vi "Unflatten pcap CAN to XNET CAN.vi"(6 "Offset in":i32, 8 "error in (no error)":errorcluster, 10 "pcap CAN DATA in":u8[](array[numeric]), 11 "XNET_CAN_RW in":refnum<class "XNET CAN RW.lvclass">) -> (0 "error out":errorcluster, 1 "XNET CAN Data":T1[](array[typedef]) {"payload" format="%x"; "timestamp" format="%<%.7X\n%x>T"; "type" items=["CAN Data"=0, "CAN Remote"=1, "CAN Bus Error"=2, "CAN 2.0 Data"=8, "CAN FD Data"=16, "CAN FD+BRS Data"=24, "J1939 Data"=192, "Delay"=224, "Log Trigger"=225, "Start Trigger"=226]; "identifier" format="%x"}, 2 "pcap CAN DATA out":u8[](array[numeric]), 3 "XNET_CAN_RW out":refnum<class "XNET CAN RW.lvclass">, 4 "Offset out":i32, 5 "Number Filtered":u32)   [LabVIEW 2021, in "XNET CAN RW.lvclass"]
uses:
  XNET CAN RW.lvclass
  <vilib>/xnet/xnet.llb/XNET Frame CAN.ctl
  <vilib>/xnet/xnet.llb/XNET Frame Type CAN.ctl
  C:/Program Files/National Instruments/LabVIEW 2021/vi.lib/CIF Foundation/CIF CAN RW Core/CAN_RW_CORE.lvclass
  <vilib>/CIF Foundation/CIF CAN RW Core/CAN_RW_CORE.lvclass/CAN_RW_CORE.ctl
  <vilib>/CIF Foundation/CIF PCAP Parse and Build/pcap_Parse_Build_CIF.lvclass/pcap_Parse_Build_CIF.ctl
  <vilib>/CIF Foundation/CIF CAN RW Core/Accessors/Read pcap class.vi
  <vilib>/CIF Foundation/CIF CAN RW Core/Accessors/Write pcap class.vi
  <vilib>/CIF Foundation/CIF PCAP Parse and Build/Data Accessors/Write Offset.vi
  <vilib>/CIF Foundation/CIF Utilities/Time/System Time/TAI Time to LabVIEW Time.vi
  <vilib>/CIF Foundation/CIF PCAP Parse and Build/Parse/Unflatten Packet Header.vi
  <vilib>/CIF Foundation/CIF Utilities/DataTypes/Flatten Unflatten/Unflatten U32.vi
  <vilib>/CIF Foundation/CIF PCAP Parse and Build/Utilities/Add Error.vi
  <vilib>/CIF Foundation/CIF PCAP Parse and Build/Utilities/Add Error Core.vi
  <vilib>/CIF Foundation/CIF PCAP Parse and Build/pcap_Parse_Build_CIF.lvclass
  <vilib>/CIF Foundation/CIF CAN RW Core/CAN_RW_CORE.lvclass
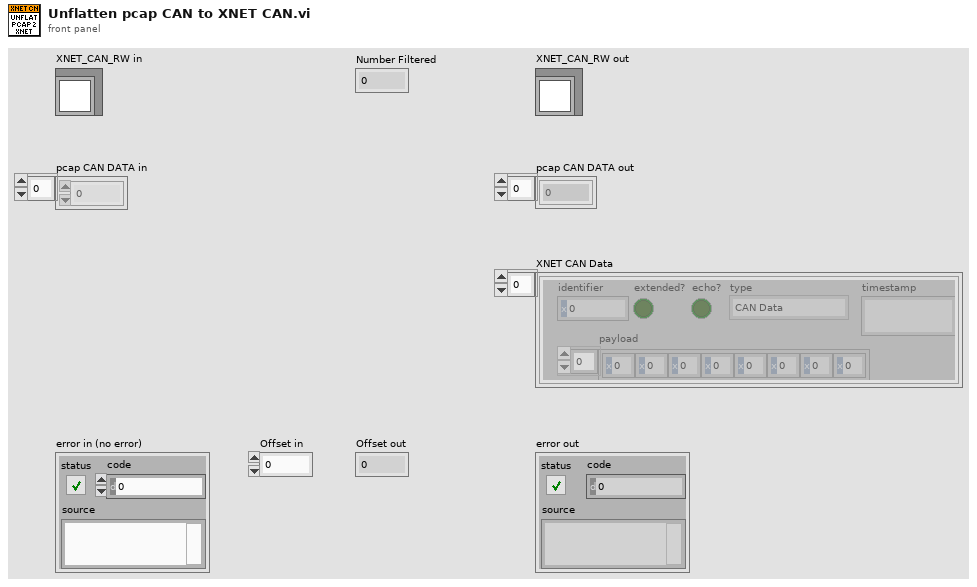
[diagram p1: front panel]
types:
  T1 = typedef "XNET Frame CAN.ctl" = cluster{"timestamp":timestamp, "payload":u8[], "identifier":u32, "type":T2, "extended?":bool, "echo?":bool}
  T2 = typedef "XNET Frame Type CAN.ctl" = u8
  T3 = typedef "pcap_Parse_Build_CIF.lvclass/Socket CAN Header.ctl" = cluster{"CANID and Flags":u32, "Payload Length":u8, "FD Flags":u8, "RSVD":u8, "Len8 DLC":u8}
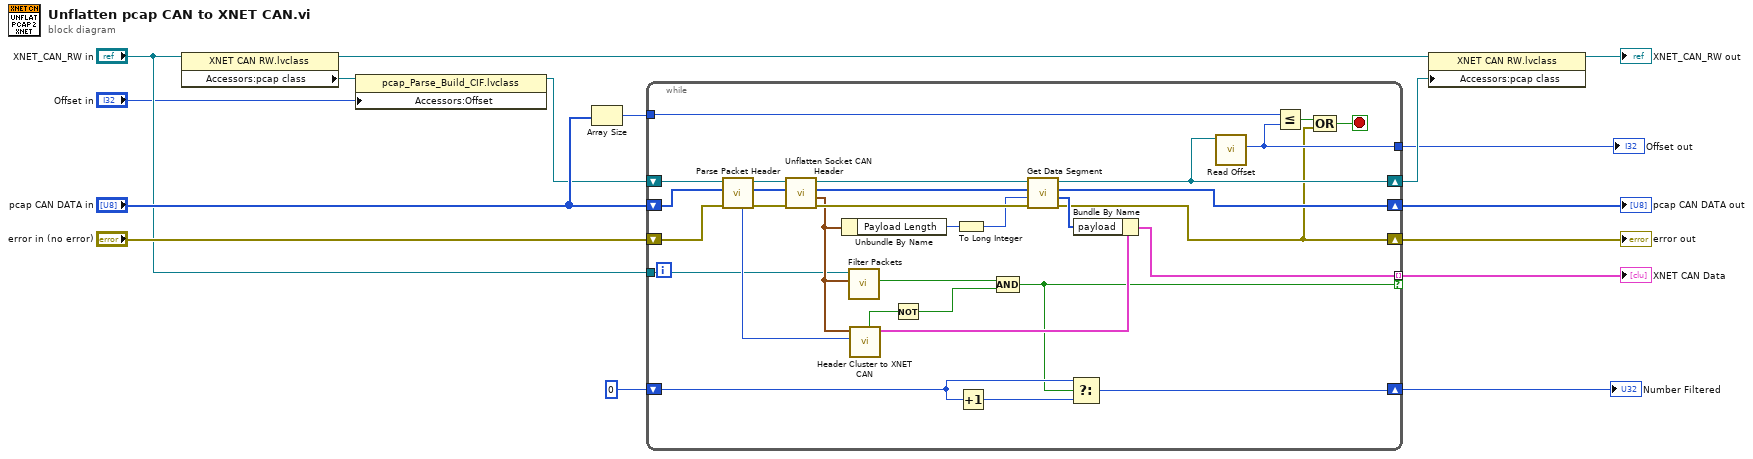
[diagram p0: block diagram]
diagram:
  n1 = property class="XNET CAN RW.lvclass"(reference="XNET_CAN_RW in") -> (reference out=w7:refnum<class "XNET CAN RW.lvclass">, "Accessors:pcap class"=w6:refnum<class "pcap_Parse_Build_CIF.lvclass">)  [unwired: 1 in, 1 out]
  n2 = property class="pcap_Parse_Build_CIF.lvclass"(reference=w6, "Accessors:Offset"="Offset in") -> (reference out=w4:refnum<class "pcap_Parse_Build_CIF.lvclass">)  [unwired: 1 in, 1 out]
  n3 = Array Size(array="pcap CAN DATA in") -> (size(s)=w11:i32)
  n4 = while {
    shift-right: [w18] -> w16
    shift-left: "error in (no error)" -> [w45]
    shift-right: [w37] -> w13
    shift-left: "pcap CAN DATA in" -> [w46]
    shift-right: [w30] -> w9
    shift-left: w4 -> [w47]
    tunnel: [w32] -> w14 mode=indexing if=w21
    tunnel: w11 -> [w29]
    tunnel: "XNET_CAN_RW in" -> [w27]
    tunnel: [w24] -> w3
    shift-right: [w20] -> w1
    shift-left: u32 0 -> [w22]
    stop <- w17 stop-if-true
    n5 = call <vilib>:"Parse Packet Header.vi"("error in (no error)"=w45, "Bytes in"=w46, "pcap Parse and Build in"=w47) -> ("error out"=w42:errorcluster, "Bytes out"=w43:u8[], "pcap Parse and Build out"=w44:refnum<class "pcap_Parse_Build_CIF.lvclass">, "TAI Time (ns)"=w41:i64)  [unwired: 3 in, 2 out]
    n6 = call <vilib>:"Unflatten Socket CAN Header.vi"("error in (no error)"=w42, "Bytes in"=w43, "pcap Parse and Build in"=w44) -> ("error out"=w36:errorcluster, "Socket CAN Header"=w28:T3, "Bytes out"=w38:u8[], "pcap Parse and Build out"=w39:refnum<class "pcap_Parse_Build_CIF.lvclass">)  [unwired: 5 in]
    n7 = Unbundle By Name(w28) -> ("Payload Length"=w35:u8)
    n8 = call <vilib>:"Filter Packets.vi"("CAN Header in"=w28, "CAN_RW_CORE"=w27) -> ("Valid"=w26:bool)  [unwired: 9 in]
    n9 = call "Header Cluster to XNET CAN.vi"("TAI Time (ns)"=w41, "Socket CAN Header"=w28) -> ("XNET CAN frame"=w40:T1, "Unsupported"=w31:bool)  [unwired: 8 in]
    n10 = Not(x=w31) -> (.not. x?=w25:bool)
    n11 = To Long Integer(number=w35) -> (32bit integer=w34:i32)
    n12 = Increment(x=w22) -> (x+1=w23:u32)
    n13 = Compound Arithmetic op=AND(w26, w25) -> (w21:bool)
    n14 = call <vilib>:"Get Data Segment.vi"("error in (no error)"=w36, "Length"=w34, "Bytes in"=w38, "pcap Parse and Build in"=w39) -> ("error out"=w18:errorcluster, "Data Segment"=w33:u8[], "Bytes out"=w37:u8[], "pcap Parse and Build out"=w30:refnum<class "pcap_Parse_Build_CIF.lvclass">)  [unwired: 4 in]
    n15 = Select(t=w22, s=w21, f=w23) -> (s? t:f=w20:u32)
    n16 = Bundle By Name(cluster=w40, "payload"=w33) -> (w32:T1)
    n17 = call <vilib>:"Read Offset.vi"("pcap Parse and Build in"=w30) -> ("Offset"=w24:i32)  [unwired: 8 in, 2 out]
    n18 = Less Or Equal?(x=w29, y=w24) -> (x <= y?=w19:bool)
    n19 = Compound Arithmetic op=OR(w19, w18) -> (w17:bool)
  }
  "error out" <- w16
  "pcap CAN DATA out" <- w13
  "XNET CAN Data" <- w14
  "Number Filtered" <- w1
  "Offset out" <- w3
  n20 = property class="XNET CAN RW.lvclass"(reference=w7, "Accessors:pcap class"=w9) -> (reference out=→"XNET_CAN_RW out":refnum<class "XNET CAN RW.lvclass">)  [unwired: 1 in, 1 out]
